vi "NT Server.vi"(7 "Logging Config":T1={"Enable"=FALSE, "Log Path"=path "", "Log Flush (s)"=0.25}, 8 "error in (no error)":errorcluster, 9 "preloads":string[](array[string])=[""]) -> (0 "error out":errorcluster)   [LabVIEW 2023]
doc: "This VI starts the Network Table services for the robot. The top level of Robot Main is a good location for this.\nYou may then read and write variables and they will be shared with Network Table clients.\nIf you enable logging, NT writes will still be shared to dashboards periodically, and all writes will be logged to on-robot wpilog files."
uses:
  <vilib>/Rock Robotics/Network Tables/NT Globals.vi
  FRC_NetworkTablesLV.so
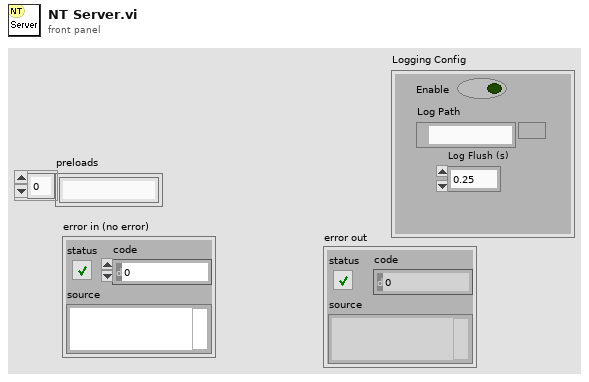
[diagram p1: front panel]
types:
  T1 = cluster{"Enable":bool, "Log Path":path, "Log Flush (s)":dbl}
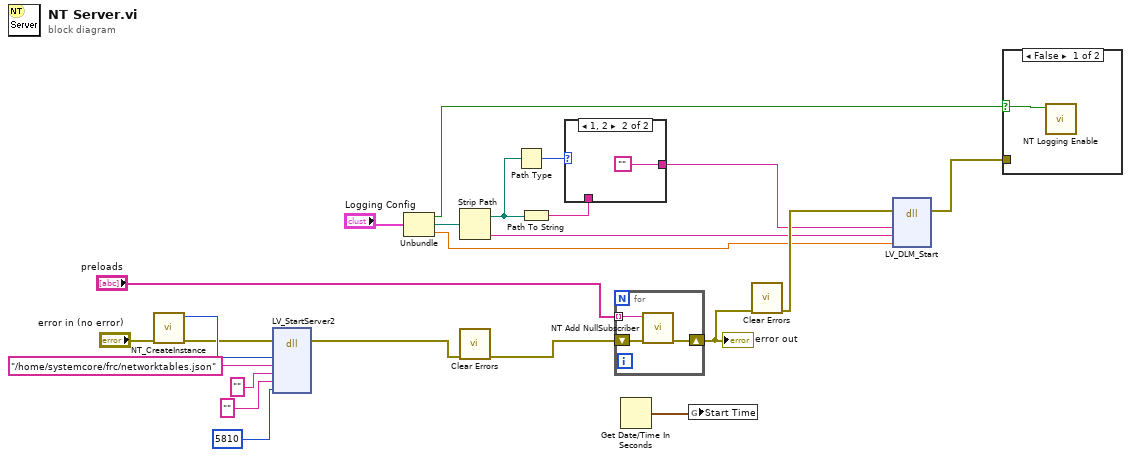
[diagram p0: block diagram]
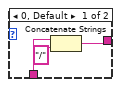
[diagram p3: hidden frame]
diagram:
  n1 = call <vilib>:"NT_CreateInstance.vi"("error in (no error)"="error in (no error)") -> ("error out"=w19:errorcluster, "InstanceHandle"=w23:u64)  [unwired: 9 in]
  n2 = dll-call lib="FRC_NetworkTablesLV.*" fn="LV_StartServer2"(error in=w19, "InstHandle"=w23, "persistFileName"="/home/systemcore/frc/networktables.json", "listenAddr"="", "mdnsSvc"="", "port4"=u16 5810 ("port")) -> (error out=w14:errorcluster)  [unwired: 8 in, 1 out]
  n3 = Unbundle("Logging Config") -> ("Enable"=w7:bool, "Log Path"=w10:path, "Log Flush (s)"=w9:dbl)
  n4 = Strip Path(path=w10) -> (stripped path=w6:path, name=w8:string)
  n5 = call <vilib>:"Clear Errors.vi"("error in (no error)"=w14) -> ("error out"=w16:errorcluster)  [unwired: 5 in, 1 out]
  n6 = Path Type(1:w6) -> (0:w5:i16)
  n7 = Path To String(path=w6) -> (string=w4:string)
  n8 = case shown="1, 2" w5 {
    tunnel: [w24 ""] -> w3
    tunnel: w4 -> [w26 _]
    frame 0, Default {
      n9 = Concatenate Strings(w26, "/" ("string")) -> (w24:string)
    }
    frame 1, 2 {
    }
  }
  n10 = for {
    shift-right: [w29] -> w13
    shift-left: w16 -> [w30]
    tunnel: "preloads" -> [w28] mode=indexing
    n11 = call <vilib>:"NT Add NullSubscriber.vi"("error in (no error)"=w30, "match Pattern"=w28) -> ("error out"=w29:errorcluster)  [unwired: 9 in]
  }
  "error out" <- w13
  n12 = Get Date/Time In Seconds() -> (seconds since 1Jan1904=w17:timestamp)
  n13 = global write "NT Globals.vi" "Start Time"(w17) -> ()
  n14 = call <vilib>:"Clear Errors.vi"("error in (no error)"=w13) -> ("error out"=w12:errorcluster)  [unwired: 5 in, 1 out]
  n15 = dll-call lib="FRC_NetworkTablesLV.*" fn="LV_DLM_Start"(error in=w12, "dir"=w3, "name"=w8, "period(s)"=w9) -> (error out=w2:errorcluster)  [unwired: 6 in, 1 out]
  n16 = case shown="False" w7 {
    selector: w7 -> [w31 _]
    tunnel: w2 -> [_ _]
    frame False {
      n17 = call <vilib>:"NT Logging Enable.vi"("Enable"=w31) -> ()  [unwired: 11 in]
    }
    frame True {
      # "default is on"
    }
  }
